vi "wiringPiI2CWriteBlockData.vi"(8 "error in (no error)":errorcluster, 9 "values":u8[](array[numeric]), 10 "reg":i32, 11 "devID":T1) -> (0 "error out":errorcluster, 3 "return":i32)   [LabVIEW 2020, in "wiringPi.lvlib"]
doc: "<b>_______________________________________________________________</b>\n** Author: Juan José Villacorta\n** LabVIEW wrapper for C library <b> wiringPi </b>,\n** https://github.com/WiringPi/WiringPi\n<b>_______________________________________________________________</b>\n\n/*\n * wiringPiI2CReadReg8: wiringPiI2CReadReg16:\n * Write a block of data to the given register\n *********************************************************************************\n */"
uses:
  wiringPi.lvlib
  Type Defs/I2C Device.ctl
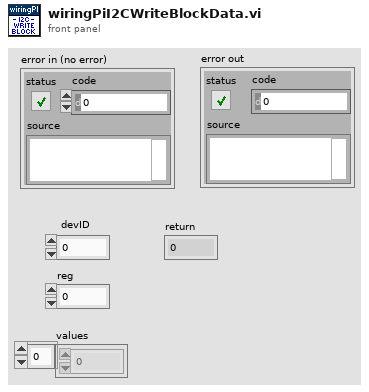
[diagram p1: front panel]
types:
  T1 = typedef "wiringPi.lvlib/I2C Device.ctl" = i32
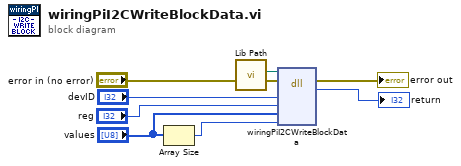
[diagram p0: block diagram]
diagram:
  n1 = Array Size(array="values") -> (size(s)=w1:i32)
  n2 = call "Lib Path.vi"() -> ("path out"=w6:path)  [unwired: 11 in]
  n3 = dll-call lib="libLVwiringPI.so" fn="wiringPiI2CWriteBlockData"(path in=w6, error in="error in (no error)", "fd"="devID", "reg"="reg", "values"="values", "size"=w1) -> (error out=→"error out":errorcluster, "return type"=→"return":i32)  [unwired: 5 in, 1 out]
